vi "Pop.vi"(8 "error in (no error)":errorcluster, 11 "Navigator in":refnum<class "Navigator.lvclass">) -> (0 "error out":errorcluster, 3 "Navigator out":refnum<class "Navigator.lvclass">)   [LabVIEW 2024, in "Navigator.lvclass"]
doc: "Remove last route from Navigator stack."
uses:
  Navigator.lvclass
  Navigator.lvclass/Navigator.ctl
  NavigatableView/NavigatableView.lvclass
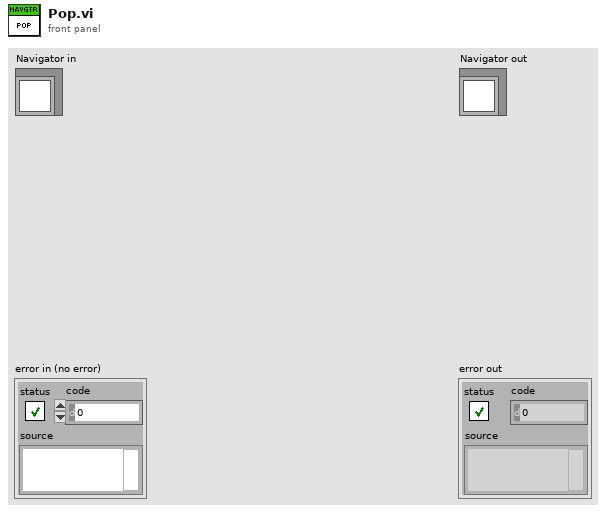
[diagram p1: front panel]
types:
  T1 = typedef "Navigator.lvclass/Route.ctl" = cluster{"Name":string, "Path":path, "Builder":refnum<class "NavigatableView.lvclass">}
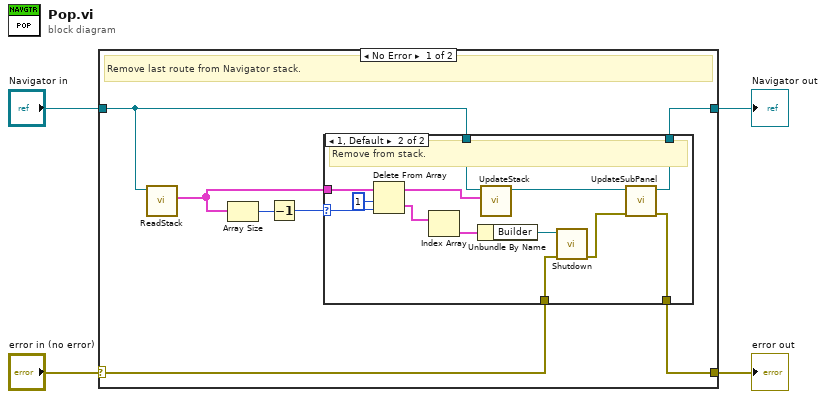
[diagram p0: block diagram]
diagram:
  n1 = case shown="No Error" "error in (no error)" {
    selector: "error in (no error)" -> [w9 w28]
    tunnel: [w8 w28] -> w1
    tunnel: [w10 w27] -> w4
    tunnel: "Navigator in" -> [w6 w27]
    frame No Error {
      # "Remove last route from Navigator stack."
      n2 = call "ReadStack.vi"("Navigator in"=w6) -> ("Stack"=w5:T1[])  [unwired: 8 in, 2 out]
      n3 = Array Size(array=w5) -> (size(s)=w11:i32)
      n4 = Decrement(x=w11) -> (x-1=w7:i32)
      n5 = case shown="1, Default" w7 {
        selector: w7 -> [_ w24]
        tunnel: w5 -> [_ w25]
        tunnel: w6 -> [w12 w16]
        tunnel: [w12 w21] -> w10
        tunnel: w9 -> [w13 w19]
        tunnel: [w13 w20] -> w8
        frame 0 {
          # "Never have empty stack."
        }
        frame 1, Default {
          # "Remove from stack."
          n6 = Delete From Array(array=w25, length=1, index=w24) -> (deleted portion=w23:T1[], array with subset deleted=w14:T1[])
          n7 = Index Array(array=w23) -> (element=w22:T1)  [unwired: 1 in]
          n8 = Unbundle By Name(w22) -> ("Builder"=w18:refnum<class "NavigatableView.lvclass">)
          n9 = call "UpdateStack.vi"("Stack"=w14, "Navigator in"=w16) -> ("Navigator out"=w15:refnum<class "Navigator.lvclass">)  [unwired: 8 in, 1 out]
          n10 = call-dynamic "Shutdown.vi"("error in (no error)"=w19, "NavigatableView in"=w18) -> ("error out"=w17:errorcluster)  [unwired: 8 in, 1 out]
          n11 = call "UpdateSubPanel.vi"("error in (no error)"=w17, "Navigator in"=w15) -> ("error out"=w20:errorcluster, "Navigator out"=w21:refnum<class "Navigator.lvclass">)  [unwired: 8 in]
        }
      }
    }
    frame Error {
    }
  }
  "error out" <- w1
  "Navigator out" <- w4
